vi "configure_train_parameters.vi"(4 "Fs":dbl=50000.0 min=0.0 max=50000.0, 5 "Amplitude Step":dbl, 6 "Frequency":dbl, 7 "Current Type":enum32{"Constant", "Staircase"}(tab), 8 "error in":errorcluster, 9 "NumCycles":u16, 10 "Pulse width":dbl, 11 "Amplitude":dbl) -> (0 "error out":errorcluster, 3 "Output train":waveform(dbl)(graph))   [LabVIEW 2025, in "tSNIP.lvlib"]
uses:
  tSNIP.lvlib
  <vilib>/Waveform/WDTOps.llb/WDT Append Waveforms DBL.vi
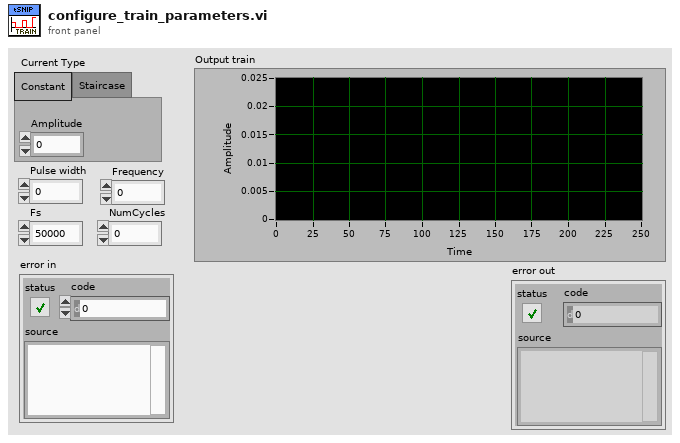
[diagram p1: front panel]
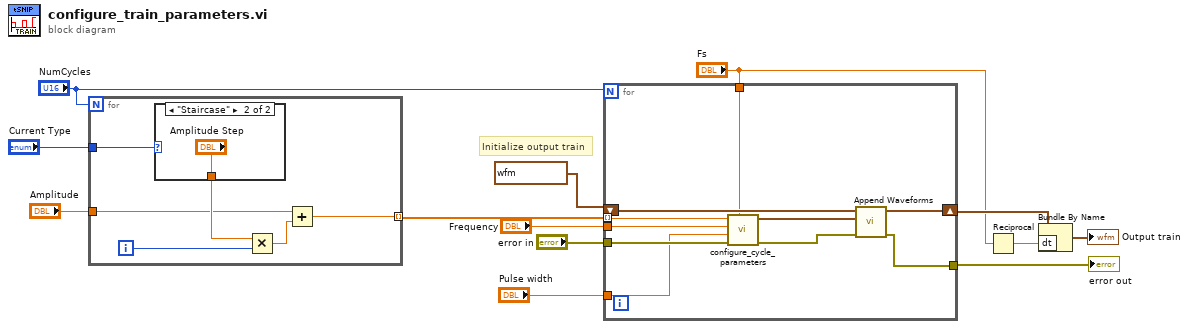
[diagram p0: block diagram]
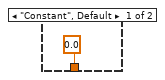
[diagram p2: hidden frame]
diagram:
  # "Initialize output train"
  n1 = for {
    N: "NumCycles" -> [_]
    tunnel: "Amplitude" -> [w17]
    tunnel: [w15] -> w4 mode=indexing
    tunnel: "Current Type" -> [w14]
    i -> [w18]
    n2 = case shown="\"Staircase\"" w14 {
      tunnel: [0.0 ("Amplitude Step") "Amplitude Step"] -> w19
      frame "Constant", Default {
      }
      frame "Staircase" {
      }
    }
    n3 = Multiply(x=w19, y=w18) -> (x*y=w16:dbl)
    n4 = Add(x=w17, y=w16) -> (x+y=w15:dbl)
  }
  n5 = for {
    N: "NumCycles" -> [_]
    shift-right: [w31] -> w12
    shift-left: waveform(dbl) {"t0"=timestamp(0 s since 1904-01-01), "dt"=1.0, "Y"=[]} ("waveform out") -> [w28]
    tunnel: "error in" -> [w30]
    tunnel: "Fs" -> [w26]
    tunnel: [w25] -> w8
    tunnel: "Frequency" -> [w24]
    tunnel: w4 -> [w23] mode=indexing
    tunnel: "Pulse width" -> [w22]
    n6 = call "configure_cycle_parameters.vi"("Fs"=w26, "error in"=w30, "Pulse width"=w22, "Frequency"=w24, "Amplitude"=w23) -> ("error out"=w29:errorcluster, "output cycle"=w27:waveform(dbl))  [unwired: 5 in]
    n7 = call-poly <vilib>:"Append Waveforms.vi"("error in (no error)"=w29, "waveform B"=w27, "waveform A"=w28) -> ("error out"=w25:errorcluster, "waveform out"=w31:waveform(dbl))  [unwired: 7 in]
  }
  "error out" <- w8
  n8 = Reciprocal(x="Fs") -> (1/x=w11:dbl)
  n9 = Bundle By Name(cluster=w12, "dt"=w11) -> (→"Output train":waveform(dbl))
